vi "PathPlanner_RotationTarget_FromJSON.vi"(11 "JSON String":string) -> (0 "Exists":bool=TRUE, 3 "RotationTargets":T2[](array[typedef]) {"rotation"."SIN" format="%13.4f"; "rotation"."COS" format="%13.4f"; "rotation"."VALUE" format="%13.4f"})   [LabVIEW 2019, in "PathPlanner24.lvlib"]
doc: "Create a rotation target from json\n \nInputs: \n - JSON String - string - string potentially containing one or more of rotation target\n\nOutputs:\n - RotationTarget - array - Set of rotation targets defined by the given json string\n - Exists - boolean - TRUE if any rotation targets were found in the JSON string."
uses:
  PathPlanner24.lvlib
  TypeDef/PathPlannerRotationTarget.ctl
  <vilib>/Rock Robotics/WPI/ThirdParty/JAS_Junk/TrajLib/TypeDef/ROTATION2D.ctl
  <vilib>/Rock Robotics/WPI/ThirdParty/JAS_Junk/TrajLib/Conv_Deg_Radians.vi
  <vilib>/Rock Robotics/WPI/ThirdParty/JAS_Junk/TrajLib/Rotation2d_CreateAngle.vi
  <vilib>/Rock Robotics/WPI/ThirdParty/JAS_Junk/TrajLib/Trajectory_Library.lvlib
panel:
  in  "rotationTargets":T1(array[cluster])
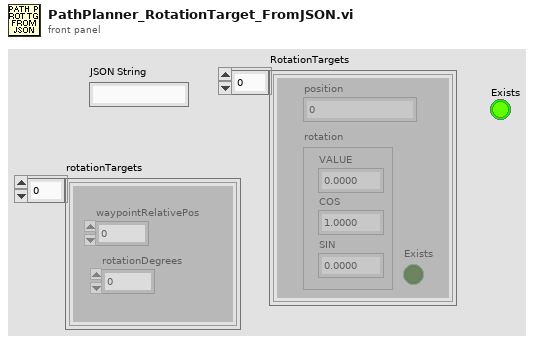
[diagram p1: front panel]
types:
  T1 = cluster{"waypointRelativePos":dbl, "rotationDegrees":dbl}[]
  T2 = typedef "PathPlanner24.lvlib/PathPlannerRotationTarget.ctl" = cluster{"position":dbl, "rotation":T3, "Exists":bool}
  T3 = typedef "Trajectory_Library.lvlib/ROTATION2D.ctl" = cluster{"VALUE":dbl, "COS":dbl, "SIN":dbl}
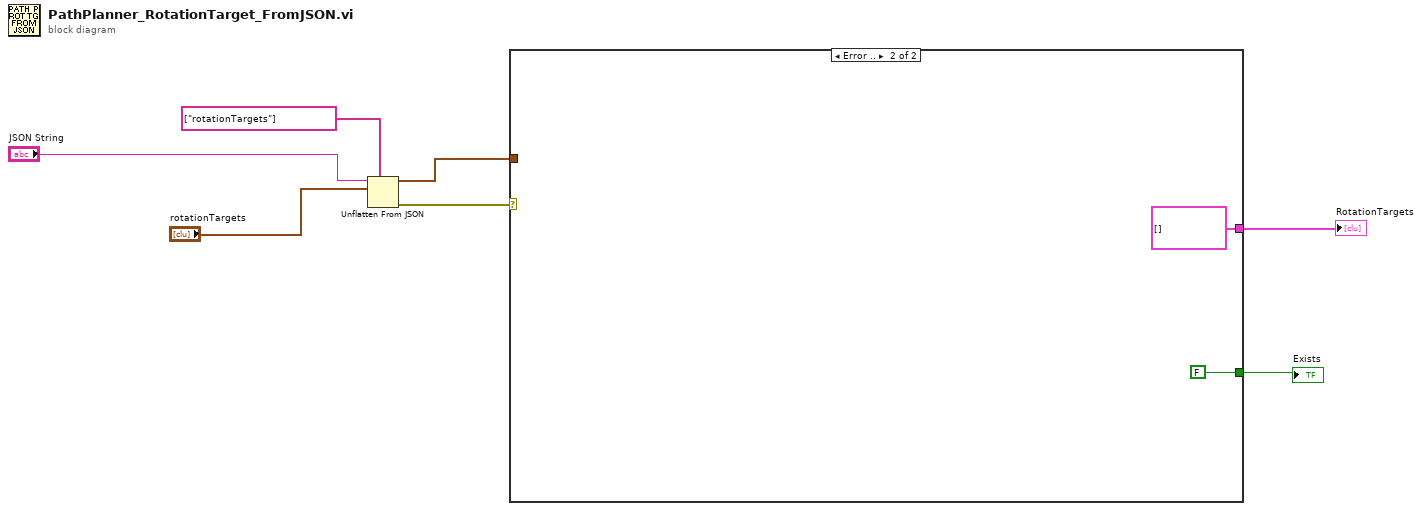
[diagram p0: block diagram]
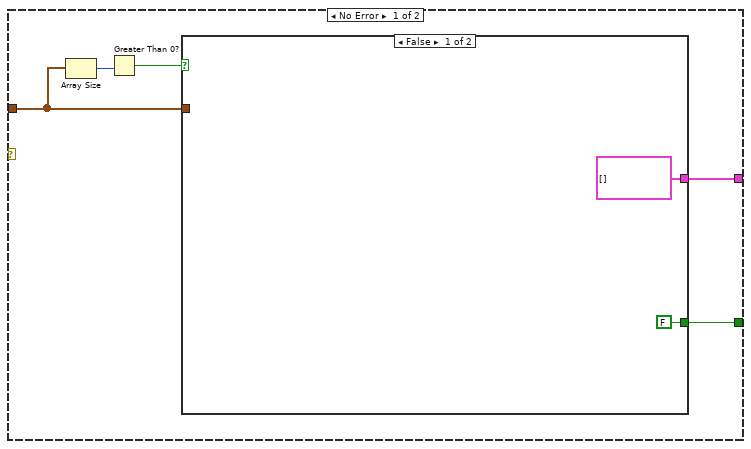
[diagram p2: hidden frame]
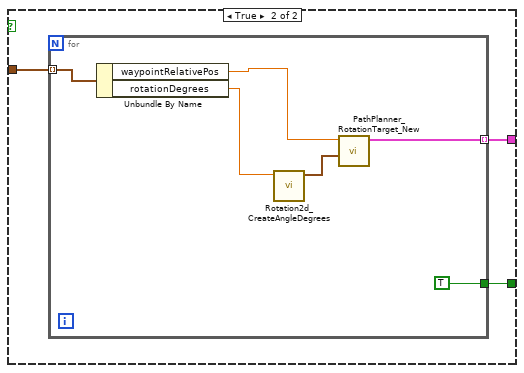
[diagram p3: hidden frame]
diagram:
  n1 = Unflatten From JSON(path=string[] ["rotationTargets"] ("path 7"), JSON string="JSON String", type and defaults="rotationTargets") -> (value=w3:T1, error out=w4:errorcluster)  [unwired: 4 in]
  n2 = case shown="Error .." w4 {
    tunnel: w3 -> [w10 _]
    tunnel: [w9 T2[] []] -> w2
    tunnel: [w8 FALSE] -> w1
    frame No Error {
      n3 = Array Size(array=w10) -> (size(s)=w12:i32)
      n4 = Greater Than 0?(x=w12) -> (x > 0?=w11:bool)
      n5 = case shown="False" w11 {
        tunnel: w10 -> [_ w17]
        tunnel: [T2[] [] w16] -> w9
        tunnel: [FALSE w15] -> w8
        frame False {
        }
        frame True {
          n6 = for {
            tunnel: w17 -> [w23] mode=indexing
            tunnel: [w19] -> w16 mode=indexing
            tunnel: [TRUE] -> w15
            n7 = Unbundle By Name(w23) -> ("waypointRelativePos"=w22:dbl, "rotationDegrees"=w21:dbl)
            n8 = call <vilib>:"Rotation2d_CreateAngleDegrees.vi"("Angle_Degrees"=w21) -> ("ROTATION"=w20:T3)  [unwired: 10 in]
            n9 = call "PathPlanner_RotationTarget_New.vi"("rotation"=w20, "position"=w22) -> ("RotationTarget"=w19:T2)  [unwired: 9 in]
          }
        }
      }
    }
    frame Error {
    }
  }
  "RotationTargets" <- w2
  "Exists" <- w1
